vi "Parse Set Path.vi"(8 "error in (no error)":errorcluster caption="에러 입력(에러 없음)", 10 "JSON string":string, 11 "Instrument Manager 입력":refnum<class "Instrument Manager.lvclass">) -> (0 "error out":errorcluster caption="에러 출력", 1 "Filter path":T1, 2 "Input path":T2, 3 "Instrument Manager 출력":refnum<class "Instrument Manager.lvclass">, 5 "Set Path Param":T3)   [LabVIEW 2023, in "Instrument Manager.lvclass"]
uses:
  Instrument Manager.lvclass
  Param Definition/Set Path Param.ctl
  Module/CE RF Switch Box/Type Definition/Input path.ctl
  Module/CE RF Switch Box/Type Definition/Filter path.ctl
  Instrument Manager.lvclass/Instrument Manager.ctl
  Module/CE RF Switch Box/RF Switch Box.lvlib
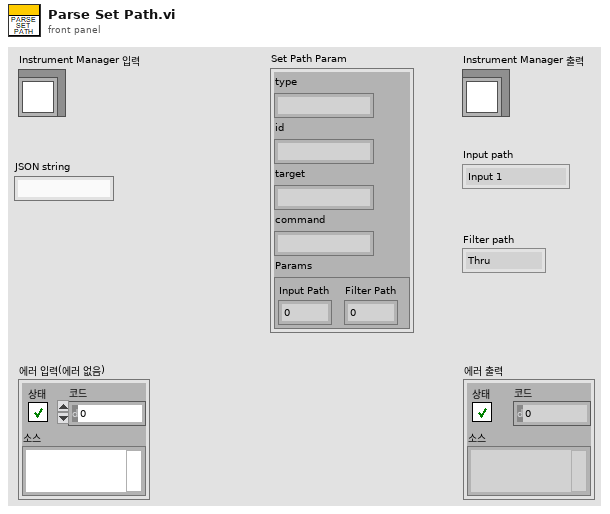
[diagram p1: front panel]
types:
  T1 = typedef "RF Switch Box.lvlib/Filter path.ctl" = enum16{"Thru", "Direct Amp", "1G HPF", "3G HPF", "7G HPF", "6G HPF", "port 1", "port 2", "port 3", "port 4", "port 5", "port 6", "port 7", "port 8", "port 9", "port 10", "port 11", "port 12", "port 13", "port 14", "port 15", "port 16", "port 17", "port 18"}
  T2 = typedef "RF Switch Box.lvlib/Input path.ctl" = enum16{"Input 1", "Input 2", "Input 3"}
  T3 = typedef "Instrument Manager.lvclass/Set Path Param.ctl" = cluster{"type":string, "id":string, "target":string, "command":string, "Params":cluster{"Input Path":i32, "Filter Path":i32}}
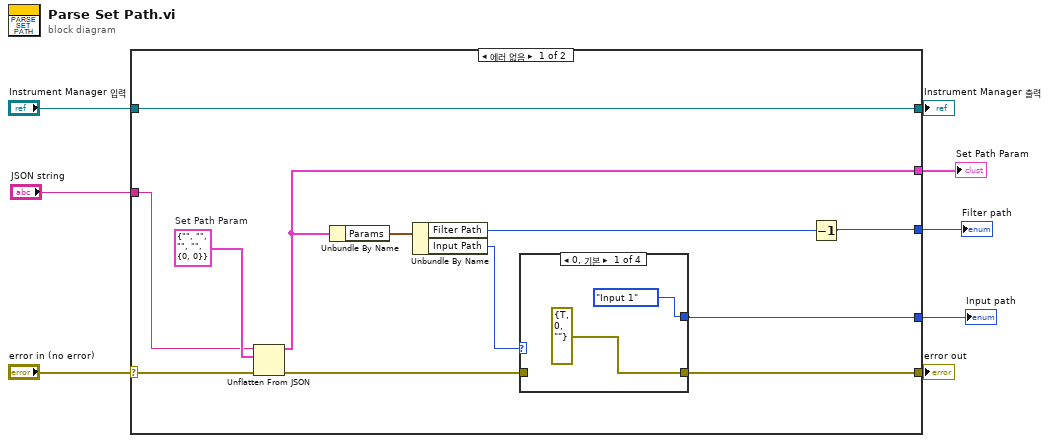
[diagram p0: block diagram]
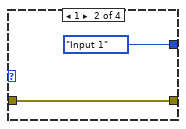
[diagram p2: hidden frame]
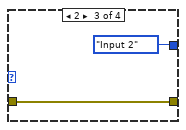
[diagram p3: hidden frame]
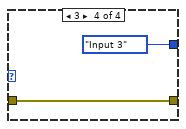
[diagram p4: hidden frame]
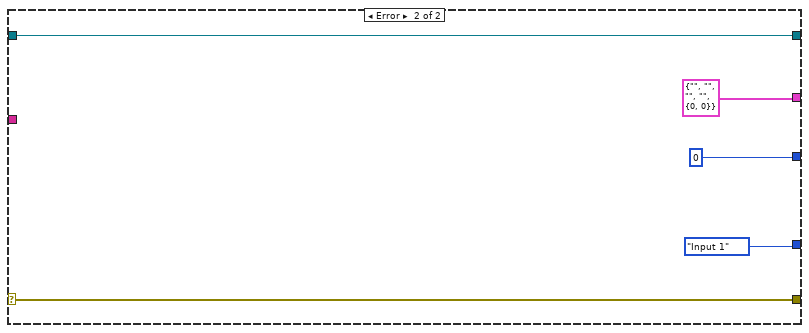
[diagram p5: hidden frame]
diagram:
  n1 = case shown="에러 없음" "error in (no error)" {
    selector: "error in (no error)" -> [w19 w33]
    tunnel: [w15 w33] -> w7
    tunnel: [w20 w32] -> w5
    tunnel: "Instrument Manager 입력" -> [w20 w32]
    tunnel: "JSON string" -> [w17 _]
    tunnel: [w11 T3 {"type"="", "id"="", "target"="", "command"="", "Params"={"Input Path"=0, "Filter Path"=0}} ("Set Path Param")] -> w3
    tunnel: [w10 0] -> w1
    tunnel: [w9 Input_path."Input 1" ("Input path")] -> w2
    frame No Error {
      w18 = T3 {"type"="", "id"="", "target"="", "command"="", "Params"={"Input Path"=0, "Filter Path"=0}}  # Set Path Param
      n2 = Unflatten From JSON(JSON string=w17, type and defaults=w18, error in (no error)=w19) -> (value=w11:T3, error out=w16:errorcluster)  [unwired: 4 in]
      n3 = Unbundle By Name(w11) -> ("Params"=w14:cluster{"Input Path":i32, "Filter Path":i32})
      n4 = Unbundle By Name(w14) -> ("Filter Path"=w12:i32, "Input Path"=w13:i32)
      n5 = case shown="0, 기본" w13 {
        tunnel: w16 -> [_ w24 w25 w27]
        tunnel: [errorcluster {"status"=TRUE, "code"=0, "source"=""} ("error out") w24 w25 w27] -> w15
        tunnel: [Input_path."Input 1" ("Input path") Input_path."Input 1" ("Input path") Input_path."Input 2" ("Input path") Input_path."Input 3" ("Input path")] -> w9
        frame 0, Default {
        }
        frame 1 {
        }
        frame 2 {
        }
        frame 3 {
        }
      }
      n6 = Decrement(x=w12) -> (x-1=w10:i32)
    }
    frame Error {
    }
  }
  "error out" <- w7
  "Instrument Manager 출력" <- w5
  "Set Path Param" <- w3
  "Input path" <- w2
  "Filter path" <- w1
